vi "xnet_canopen_destroy.vi"(8 "error in (no error)":errorcluster, 11 "xnet_co_handle":u64) -> (0 "error out":errorcluster)   [LabVIEW 2023, in "xnet_canopen.lvlib"]
uses:
  xnet_canopen.lvlib
  <vilib>/Utility/error.llb/Error Cluster From Error Code.vi
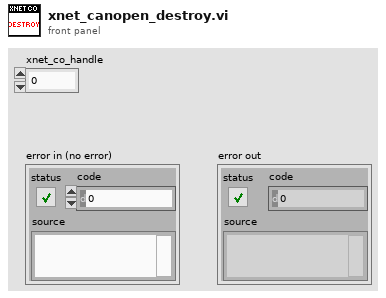
[diagram p1: front panel]
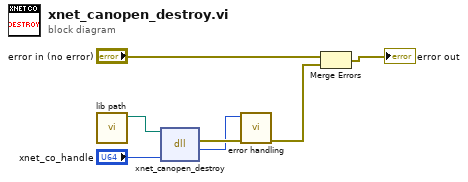
[diagram p0: block diagram]
diagram:
  n1 = call "lib path.vi"() -> ("lib path"=w6:path)  [unwired: 11 in]
  n2 = dll-call lib="?" fn="xnet_canopen_destroy"(path in=w6, "handle"="xnet_co_handle") -> (error out=w5:errorcluster, "return type"=w4:i32)  [unwired: 3 in, 1 out]
  n3 = call "error handling.vi"("error in (no error)"=w5, "return val"=w4) -> ("error out"=w7:errorcluster)  [unwired: 9 in]
  n4 = Merge Errors("error in (no error)", w7) -> (→"error out":errorcluster)
